vi "VIH ProjFile - Enum Info Array - Read.vi"(8 "error in":errorcluster, 10 "Property Name":string, 11 "XML Parent Item":refnum<k20>) -> (0 "error out":errorcluster, 1 "EnumValDscr":T1[](array[typedef]), 2 "Property found":bool, 3 "dup XML Parent Item":refnum<k20>)   [LabVIEW 2014]
doc: "::: VI Helpeks :::\nCopyright (c) 2000-2026 Konstantin Shifershteyn. All rights reserved."
uses:
  _VIH HelpGen.llb/VIH HelpGen Typedef - Cluster - Enum Value Info.ctl
  <vilib>/xml/Close Reference(Node).vi
  <vilib>/xml/Close Reference(NNMap).vi
  <vilib>/xml/NI_XML.lvlib
  <resource>/objmgr/DOMUserDefRef.rc
panel:
  # "VI Helpeks\nCopyright (c) 2012-2026 Konstantin Shifershteyn"
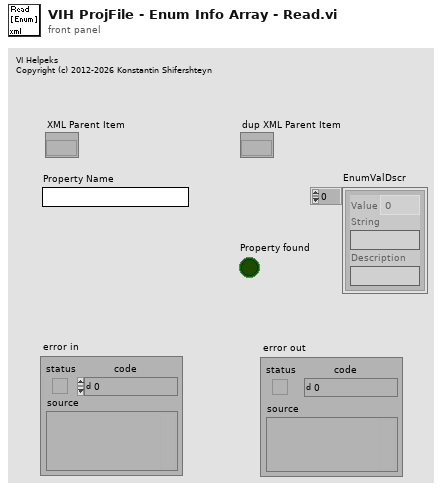
[diagram p1: front panel]
types:
  T1 = typedef "VIH HelpGen Typedef - Cluster - Enum Value Info.ctl" = cluster{"Value":ext, "String":string, "Description":string}
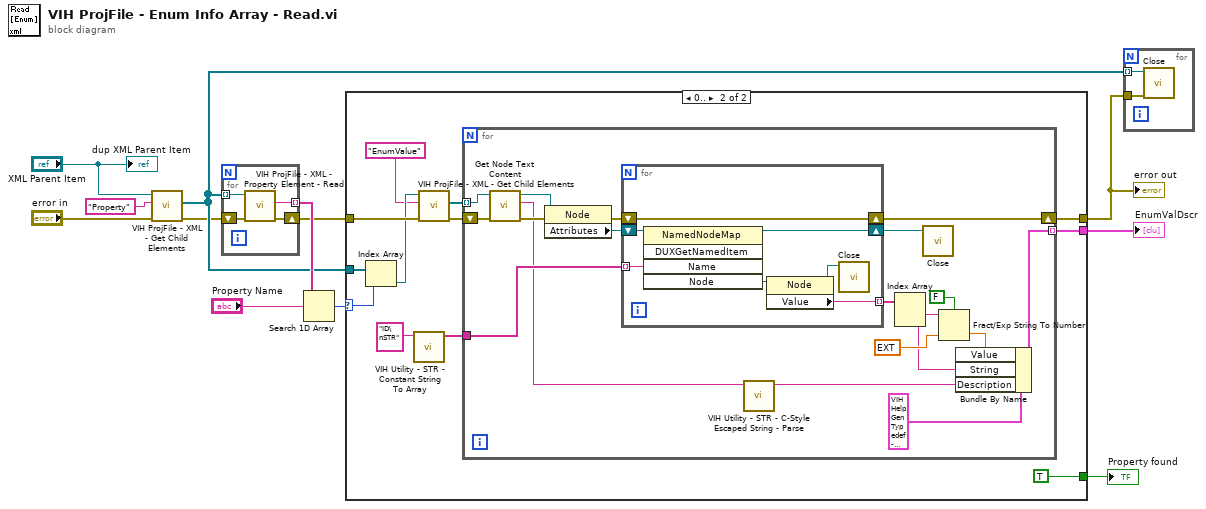
[diagram p0: block diagram]
diagram:
  n1 = call "VIH ProjFile - XML - Get Child Elements.vi"("error in"="error in", "Tag Name"="Property", "XML Parent Item"="XML Parent Item") -> ("error out"=w3:errorcluster, "Array of Elements"=w6:refnum<k20>[])  [unwired: 6 in, 1 out]
  n2 = for {
    tunnel: w6 -> [w16] mode=indexing
    shift-right: [w14] -> w10
    shift-left: w3 -> [w15]
    tunnel: [w13] -> w12 mode=indexing
    n3 = call "VIH ProjFile - XML - Property Element - Read.vi"("error in"=w15, "XML Node"=w16) -> ("error out"=w14:errorcluster, "Property Name"=w13:string)  [unwired: 6 in, 2 out]
  }
  n4 = Search 1D Array(1D array=w12, element="Property Name") -> (index of element=w11:i32)  [unwired: 1 in]
  n5 = case shown="0.." w11 {
    selector: w11 -> [_ w28]
    tunnel: [w17 w27] -> w8
    tunnel: w10 -> [w17 w26]
    tunnel: w6 -> [_ w29]
    tunnel: [_ w19] -> w9
    tunnel: [_ TRUE] -> w1
    frame ..-1 {
    }
    frame 0.. {
      n6 = Index Array(array=w29, index=w28) -> (element=w25:refnum<k20>)
      n7 = call "VIH Utility - STR - Constant String To Array.vi"("String in"="ID\nSTR") -> ("Array out"=w20:string[])  [unwired: 10 in]
      n8 = call "VIH ProjFile - XML - Get Child Elements.vi"("error in"=w26, "Tag Name"="EnumValue", "XML Parent Item"=w25) -> ("error out"=w24:errorcluster, "Array of Elements"=w23:refnum<k20>[])  [unwired: 6 in, 1 out]
      n9 = for {
        tunnel: w23 -> [w33] mode=indexing
        shift-right: [w36] -> w27
        shift-left: w24 -> [w35]
        tunnel: w20 -> [w47]
        tunnel: [w38] -> w19 mode=indexing
        n10 = call <vilib>:"Get Node Text Content.vi"("error in (no error)"=w35, "node in"=w33) -> ("error out"=w32:errorcluster, "node text"=w31:string, "node out"=w34:refnum<k20>)  [unwired: 7 in]
        n11 = property class="Node"(reference=w34, error in=w32) -> (error out=w37:errorcluster, "Attributes"=w48:refnum<k20>)  [unwired: 1 out]
        n12 = for {
          tunnel: w47 -> [w52] mode=indexing
          tunnel: [w51] -> w45 mode=indexing
          shift-right: [w50] -> w46
          shift-left: w48 -> [w55]
          shift-right: [w49] -> w36
          shift-left: w37 -> [w49]
          n13 = invoke class="NamedNodeMap" method="DUXGetNamedItem"(reference=w55, "Name"=w52) -> (reference out=w50:refnum<k20>, "Node"=w54:refnum<k20>)  [unwired: 3 in, 3 out]
          n14 = property class="Node"(reference=w54) -> (reference out=w53:refnum<k20>, "Value"=w51:string)  [unwired: 1 in, 1 out]
          n15 = call-poly <vilib>:"Close.vi"("node"=w53) -> ()  [unwired: 8 in, 1 out]
        }
        n16 = call "VIH Utility - STR - C-Style Escaped String - Parse.vi"("String in"=w31) -> ("String out"=w30:string)  [unwired: 10 in]
        n17 = Index Array(array=w45) -> (element #1=w44:string, element #2=w40:string)  [unwired: 2 in]
        n18 = call-poly <vilib>:"Close.vi"("named node map"=w46) -> ()  [unwired: 8 in, 1 out]
        n19 = Fract/Exp String To Number(use system decimal point (T)=FALSE, string=w44, default (0 dbl)=ext nan ("default (0 DBL)")) -> (number=w39:ext)  [unwired: 1 in, 1 out]
        n20 = Bundle By Name(cluster=T1 {"Value"=0.0, "String"="", "Description"=""} ("EnumValDscr (data)"), "Value"=w39, "String"=w40, "Description"=w30) -> (w38:T1)
      }
    }
  }
  "error out" <- w8
  "EnumValDscr" <- w9
  "Property found" <- w1
  n21 = for {
    tunnel: w6 -> [w57] mode=indexing
    tunnel: w8 -> [w56]
    n22 = call-poly <vilib>:"Close.vi"("error in (no error)"=w56, "node"=w57) -> ()  [unwired: 7 in, 1 out]
  }
  "dup XML Parent Item" <- "XML Parent Item"
